vi "LaneFolower.vi"() -> ()   [LabVIEW 2024]
uses:
  <vilib>/Python/Open Venv Python Session.vi
panel:
  in  "File Path":path
  in  "Lane_No.":i32
  out "ToGoLane_X":dbl[](array[numeric])=[-0.009502511471509933, -0.00958104245364666, -0.009974642656743526, -0.010631692595779896, -0.011504605412483215, -0.01254978682845831, -0.013727571815252304, -0.015002261847257614, -0.016342105343937874, -0.017719069495797157, -0.019109033048152924, -0.020491652190685272, -0.02185027115046978, -0.023171929642558098, -0.02444736659526825, -0.025670843198895454, -0.026840148493647575, -0.027956662699580193, -0.02902509644627571, -0.030053474009037018, -0.03105323575437069, -0.032038867473602295, -0.03302808105945587, -0.034041572362184525, -0.035102952271699905, -0.036238763481378555, -0.03747819736599922, -0.03885306790471077, -0.04039765149354935, -0.042148612439632416, -0.044144876301288605, -0.04642732813954353, -0.049038924276828766, -0.05202410742640495, -0.05542914569377899, -0.05930148437619209, -0.06368973851203918, -0.06864342093467712, -0.0742126852273941, -0.08044812828302383, -0.08740027993917465, -0.09511960297822952, -0.10365574806928635, -0.11305739730596542, -0.12337195128202438, -0.13464458286762238, -0.1469181925058365, -0.16023248434066772, -0.1746234893798828, -0.190122589468956]
  out "ToGpLane_Y":dbl[](array[numeric])=[0.056673385202884674, 0.06285841017961502, 0.06917627155780792, 0.07562797516584396, 0.08221480250358582, 0.08893834054470062, 0.09580045938491821, 0.10280333459377289, 0.1099495217204094, 0.11724183708429337, 0.1246834471821785, 0.13227789103984833, 0.14002907276153564, 0.14794126152992249, 0.15601910650730133, 0.16426768898963928, 0.17269249260425568, 0.18129947781562805, 0.190094992518425, 0.19908587634563446, 0.208279550075531, 0.2176838517189026, 0.22730717062950134, 0.23715846240520477, 0.24724726378917694, 0.25758373737335205, 0.2681786119937897, 0.27904340624809265, 0.290190190076828, 0.3016318380832672, 0.31338199973106384, 0.32545506954193115, 0.3378663659095764, 0.3506320118904114, 0.3637691140174866, 0.37729573249816895, 0.39123091101646423, 0.4055948555469513, 0.42040887475013733, 0.43569549918174744, 0.4514785706996918, 0.4677831828594208, 0.48463597893714905, 0.5020650625228882, 0.5201000571250916, 0.538772463798523, 0.5581153631210327, 0.5781639218330383, 0.5989552140235901, 0.620528519153595]
  out "Tracking_Err(m)":dbl=0.05746451352461557
  in  "Ld(m)":dbl=1.0 format="%#_13g"
  out "GPS_Steer_CMD(Deg)":dbl=-13.889371307932791
  out "Lane":T1(graph)=[{"Third_Lane_X"=[-0.0093022920191288, -0.009425072930753231, -0.00985750462859869, -0.010548070073127747, -0.011449389159679413, -0.012518086470663548, -0.013714795000851154, -0.015004051849246025, -0.016354387626051903, -0.01773810014128685, -0.01913149282336235, -0.020514462143182755, -0.0218708086758852, -0.023187965154647827, -0.024457033723592758, -0.025672709569334984, -0.026833219453692436, -0.027940329164266586, -0.028999147936701775, -0.03001815639436245, -0.03100910596549511, -0.031986892223358154, -0.03296966105699539, -0.03397832438349724, -0.035036876797676086, -0.03617206588387489, -0.03741329908370972, -0.03879253566265106, -0.04034423828125, -0.04210503771901131, -0.04411381483078003, -0.04641137272119522, -0.04904036968946457, -0.05204509198665619, -0.055471181869506836, -0.05936558172106743, -0.06377621740102768, -0.06875165551900864, -0.07434111088514328, -0.0805937796831131, -0.08755884319543839, -0.09528496116399765, -0.103819839656353, -0.11321000009775162, -0.12350000441074371, -0.13473232090473175, -0.14694637060165405, -0.16017811000347137, -0.17445921897888184, -0.18981638550758362], "Third_Lane_Y"=[0.056663379073143005, 0.06285057216882706, 0.06917034834623337, 0.07562372088432312, 0.08221197873353958, 0.0889367088675499, 0.09579980373382568, 0.10280342400074005, 0.10995016992092133, 0.11724283546209335, 0.124684639275074, 0.13227911293506622, 0.140030175447464, 0.14794212579727173, 0.15601962804794312, 0.16426779329776764, 0.17269212007522583, 0.18129855394363403, 0.190093532204628, 0.19908387959003448, 0.20827704668045044, 0.21768087148666382, 0.22730378806591034, 0.2371547818183899, 0.24724338948726654, 0.2575797736644745, 0.2681747376918793, 0.27903974056243896, 0.29018694162368774, 0.3016291558742523, 0.31338009238243103, 0.32545405626296997, 0.3378664553165436, 0.3506333529949188, 0.36377182602882385, 0.37729987502098083, 0.3912365734577179, 0.40560200810432434, 0.420417457818985, 0.4357053339481354, 0.4514893889427185, 0.4677945673465729, 0.4846474230289459, 0.5020757913589478, 0.520109236240387, 0.5387787818908691, 0.5581173896789551, 0.5781599283218384, 0.5989429354667664, 0.6205053329467773]}, {"Third_Lane_X"=[0.4193677306175232, 0.4193677306175232, 0.4193677306175232, 0.4193677306175232, 0.4193677306175232, 0.4193677306175232, 0.4193677306175232, 0.4193677306175232, 0.4193677306175232, 0.42097243201055806, 0.42392416776651465, 0.42498393701902, 0.4250357962365585, 0.4243763465398626, 0.4232724906954244, 0.42195267611738735, 0.42051152778688927, 0.4190382473884229, 0.4175688753060556, 0.4161152139823713, 0.4146708213415447, 0.41321472214946825, 0.41172401655332985, 0.41016610607672, 0.40850818978861925, 0.4067346649283272, 0.4047908396323909, 0.4026850775517133, 0.4003864312158304, 0.3978821262918225, 0.3951741967138616, 0.3922227445599256, 0.38908504618485606, 0.3857545290688188, 0.3822306560533131, 0.37854025974870753, 0.37470173287875413, 0.3707522348284704, 0.36670607410360523, 0.362607736842811, 0.3584846745888019, 0.35437860537888727, 0.3503258684770675, 0.3463709544143118, 0.3441532850265503, 0.3441532850265503, 0.3441532850265503, 0.3441532850265503, 0.3441532850265503, 0.3441532850265503], "Third_Lane_Y"=[0.056663379073143005, 0.06867623572446863, 0.08068909237579423, 0.09270194902711985, 0.10471480567844546, 0.11672766232977108, 0.1287405189810967, 0.1407533756324223, 0.15276623228374792, 0.16477908893507354, 0.17679194558639916, 0.18880480223772478, 0.2008176588890504, 0.21283051554037602, 0.2248433721917016, 0.23685622884302723, 0.24886908549435285, 0.2608819421456785, 0.27289479879700407, 0.2849076554483297, 0.2969205120996553, 0.30893336875098093, 0.32094622540230655, 0.33295908205363217, 0.3449719387049578, 0.3569847953562834, 0.36899765200760903, 0.3810105086589346, 0.3930233653102602, 0.40503622196158584, 0.41704907861291146, 0.4290619352642371, 0.4410747919155627, 0.4530876485668883, 0.46510050521821394, 0.47711336186953957, 0.4891262185208652, 0.5011390751721908, 0.5131519318235164, 0.525164788474842, 0.5371776451261676, 0.5491905017774932, 0.5612033584288189, 0.5732162150801444, 0.5852290717314701, 0.5972419283827957, 0.6092547850341213, 0.6212676416854469, 0.6332804983367726, 0.6452933549880981]}, {"Third_Lane_X"=[0.0, 0.0, 0.0, 0.0, 0.0, 0.0, 0.0, 0.0, 0.0, 0.0, 0.0, 0.0, 0.0, 0.0, 0.0, 0.0, 0.0, 0.0, 0.0, 0.0, 0.0, 0.0, 0.0, 0.0, 0.0, 0.0, 0.0, 0.0, 0.0, 0.0, 0.0, 0.0, 0.0, 0.0, 0.0, 0.0, 0.0, 0.0, 0.0, 0.0, 0.0, 0.0, 0.0, 0.0, 0.0, 0.0, 0.0, 0.0, 0.0, 0.0], "Third_Lane_Y"=[0.0, 0.0, 0.0, 0.0, 0.0, 0.0, 0.0, 0.0, 0.0, 0.0, 0.0, 0.0, 0.0, 0.0, 0.0, 0.0, 0.0, 0.0, 0.0, 0.0, 0.0, 0.0, 0.0, 0.0, 0.0, 0.0, 0.0, 0.0, 0.0, 0.0, 0.0, 0.0, 0.0, 0.0, 0.0, 0.0, 0.0, 0.0, 0.0, 0.0, 0.0, 0.0, 0.0, 0.0, 0.0, 0.0, 0.0, 0.0, 0.0, 0.0]}]
  out "Third_Lane_X":dbl[](array[numeric])
  out "Third_Lane_Y":dbl[](array[numeric])
  out "Second_Lane_X":dbl[](array[numeric])=[0.4193677306175232, 0.4193677306175232, 0.4193677306175232, 0.4193677306175232, 0.4193677306175232, 0.4193677306175232, 0.4193677306175232, 0.4193677306175232, 0.4193677306175232, 0.42097243201055806, 0.42392416776651465, 0.42498393701902, 0.4250357962365585, 0.4243763465398626, 0.4232724906954244, 0.42195267611738735, 0.42051152778688927, 0.4190382473884229, 0.4175688753060556, 0.4161152139823713, 0.4146708213415447, 0.41321472214946825, 0.41172401655332985, 0.41016610607672, 0.40850818978861925, 0.4067346649283272, 0.4047908396323909, 0.4026850775517133, 0.4003864312158304, 0.3978821262918225, 0.3951741967138616, 0.3922227445599256, 0.38908504618485606, 0.3857545290688188, 0.3822306560533131, 0.37854025974870753, 0.37470173287875413, 0.3707522348284704, 0.36670607410360523, 0.362607736842811, 0.3584846745888019, 0.35437860537888727, 0.3503258684770675, 0.3463709544143118, 0.3441532850265503, 0.3441532850265503, 0.3441532850265503, 0.3441532850265503, 0.3441532850265503, 0.3441532850265503]
  out "Second_Lane_Y":dbl[](array[numeric])=[0.056663379073143005, 0.06867623572446863, 0.08068909237579423, 0.09270194902711985, 0.10471480567844546, 0.11672766232977108, 0.1287405189810967, 0.1407533756324223, 0.15276623228374792, 0.16477908893507354, 0.17679194558639916, 0.18880480223772478, 0.2008176588890504, 0.21283051554037602, 0.2248433721917016, 0.23685622884302723, 0.24886908549435285, 0.2608819421456785, 0.27289479879700407, 0.2849076554483297, 0.2969205120996553, 0.30893336875098093, 0.32094622540230655, 0.33295908205363217, 0.3449719387049578, 0.3569847953562834, 0.36899765200760903, 0.3810105086589346, 0.3930233653102602, 0.40503622196158584, 0.41704907861291146, 0.4290619352642371, 0.4410747919155627, 0.4530876485668883, 0.46510050521821394, 0.47711336186953957, 0.4891262185208652, 0.5011390751721908, 0.5131519318235164, 0.525164788474842, 0.5371776451261676, 0.5491905017774932, 0.5612033584288189, 0.5732162150801444, 0.5852290717314701, 0.5972419283827957, 0.6092547850341213, 0.6212676416854469, 0.6332804983367726, 0.6452933549880981]
  out "First_Lane_Y":dbl[](array[numeric])=[0.056663379073143005, 0.06285057216882706, 0.06917034834623337, 0.07562372088432312, 0.08221197873353958, 0.0889367088675499, 0.09579980373382568, 0.10280342400074005, 0.10995016992092133, 0.11724283546209335, 0.124684639275074, 0.13227911293506622, 0.140030175447464, 0.14794212579727173, 0.15601962804794312, 0.16426779329776764, 0.17269212007522583, 0.18129855394363403, 0.190093532204628, 0.19908387959003448, 0.20827704668045044, 0.21768087148666382, 0.22730378806591034, 0.2371547818183899, 0.24724338948726654, 0.2575797736644745, 0.2681747376918793, 0.27903974056243896, 0.29018694162368774, 0.3016291558742523, 0.31338009238243103, 0.32545405626296997, 0.3378664553165436, 0.3506333529949188, 0.36377182602882385, 0.37729987502098083, 0.3912365734577179, 0.40560200810432434, 0.420417457818985, 0.4357053339481354, 0.4514893889427185, 0.4677945673465729, 0.4846474230289459, 0.5020757913589478, 0.520109236240387, 0.5387787818908691, 0.5581173896789551, 0.5781599283218384, 0.5989429354667664, 0.6205053329467773]
  out "First_Lane_X":dbl[](array[numeric])=[-0.0093022920191288, -0.009425072930753231, -0.00985750462859869, -0.010548070073127747, -0.011449389159679413, -0.012518086470663548, -0.013714795000851154, -0.015004051849246025, -0.016354387626051903, -0.01773810014128685, -0.01913149282336235, -0.020514462143182755, -0.0218708086758852, -0.023187965154647827, -0.024457033723592758, -0.025672709569334984, -0.026833219453692436, -0.027940329164266586, -0.028999147936701775, -0.03001815639436245, -0.03100910596549511, -0.031986892223358154, -0.03296966105699539, -0.03397832438349724, -0.035036876797676086, -0.03617206588387489, -0.03741329908370972, -0.03879253566265106, -0.04034423828125, -0.04210503771901131, -0.04411381483078003, -0.04641137272119522, -0.04904036968946457, -0.05204509198665619, -0.055471181869506836, -0.05936558172106743, -0.06377621740102768, -0.06875165551900864, -0.07434111088514328, -0.0805937796831131, -0.08755884319543839, -0.09528496116399765, -0.103819839656353, -0.11321000009775162, -0.12350000441074371, -0.13473232090473175, -0.14694637060165405, -0.16017811000347137, -0.17445921897888184, -0.18981638550758362]
  out "ImageString":string
  out "error out":errorcluster
  out "Python Loop Process Time":u32=33
  in  "stop":bool
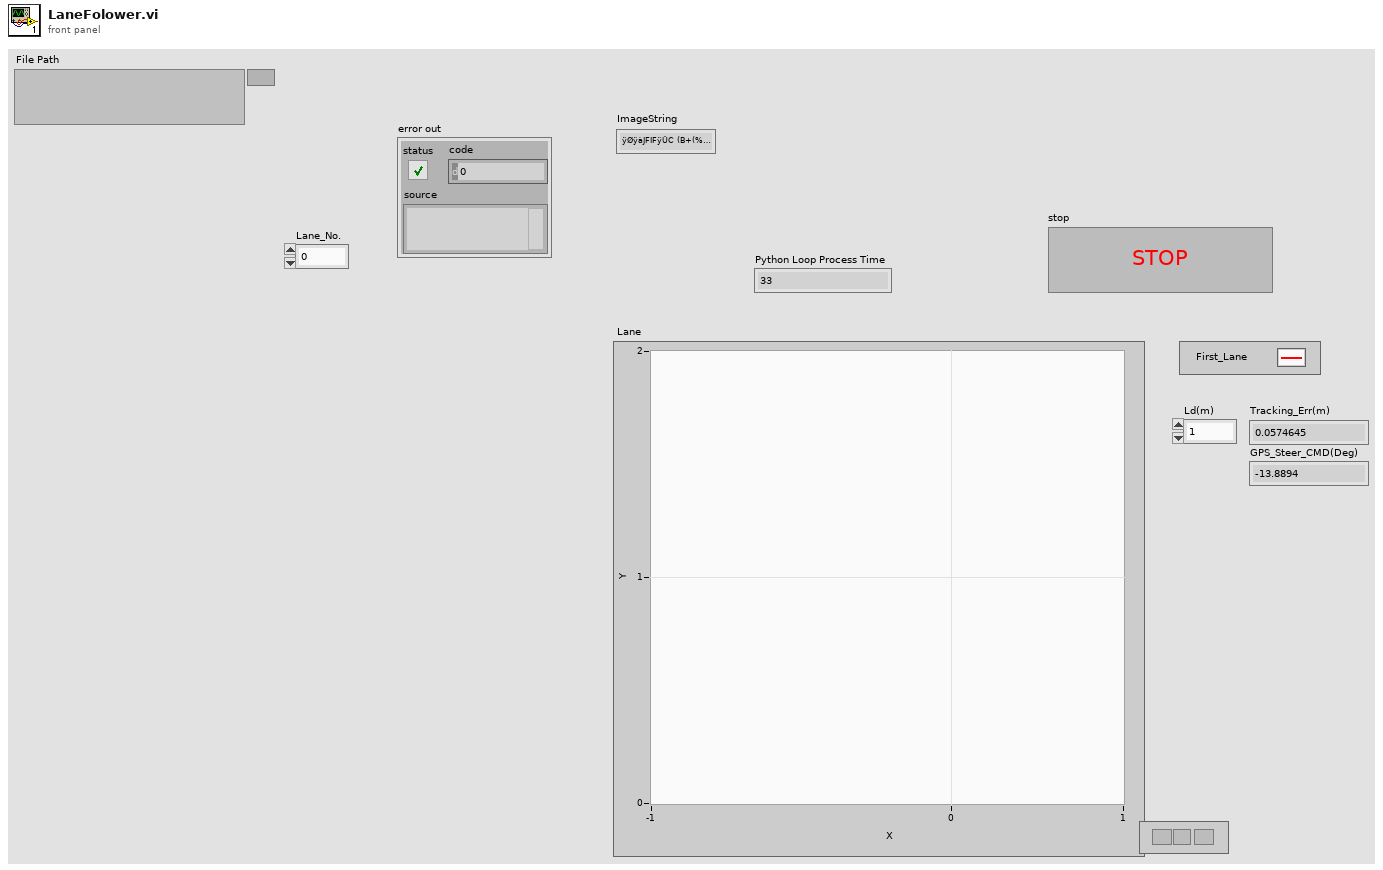
[diagram p1: front panel]
types:
  T1 = cluster{"Third_Lane_X":dbl[], "Third_Lane_Y":dbl[]}[]
  T2 = typedef "IMAQ Image.ctl" = refnum<image>
  T3 = cluster{"First_Lane_X":dbl[], "First_Lane_Y":dbl[]}
  T4 = cluster{"Second_Lane_X":dbl[], "Second_Lane_Y":dbl[]}
  T5 = cluster{"Third_Lane_X":dbl[], "Third_Lane_Y":dbl[]}
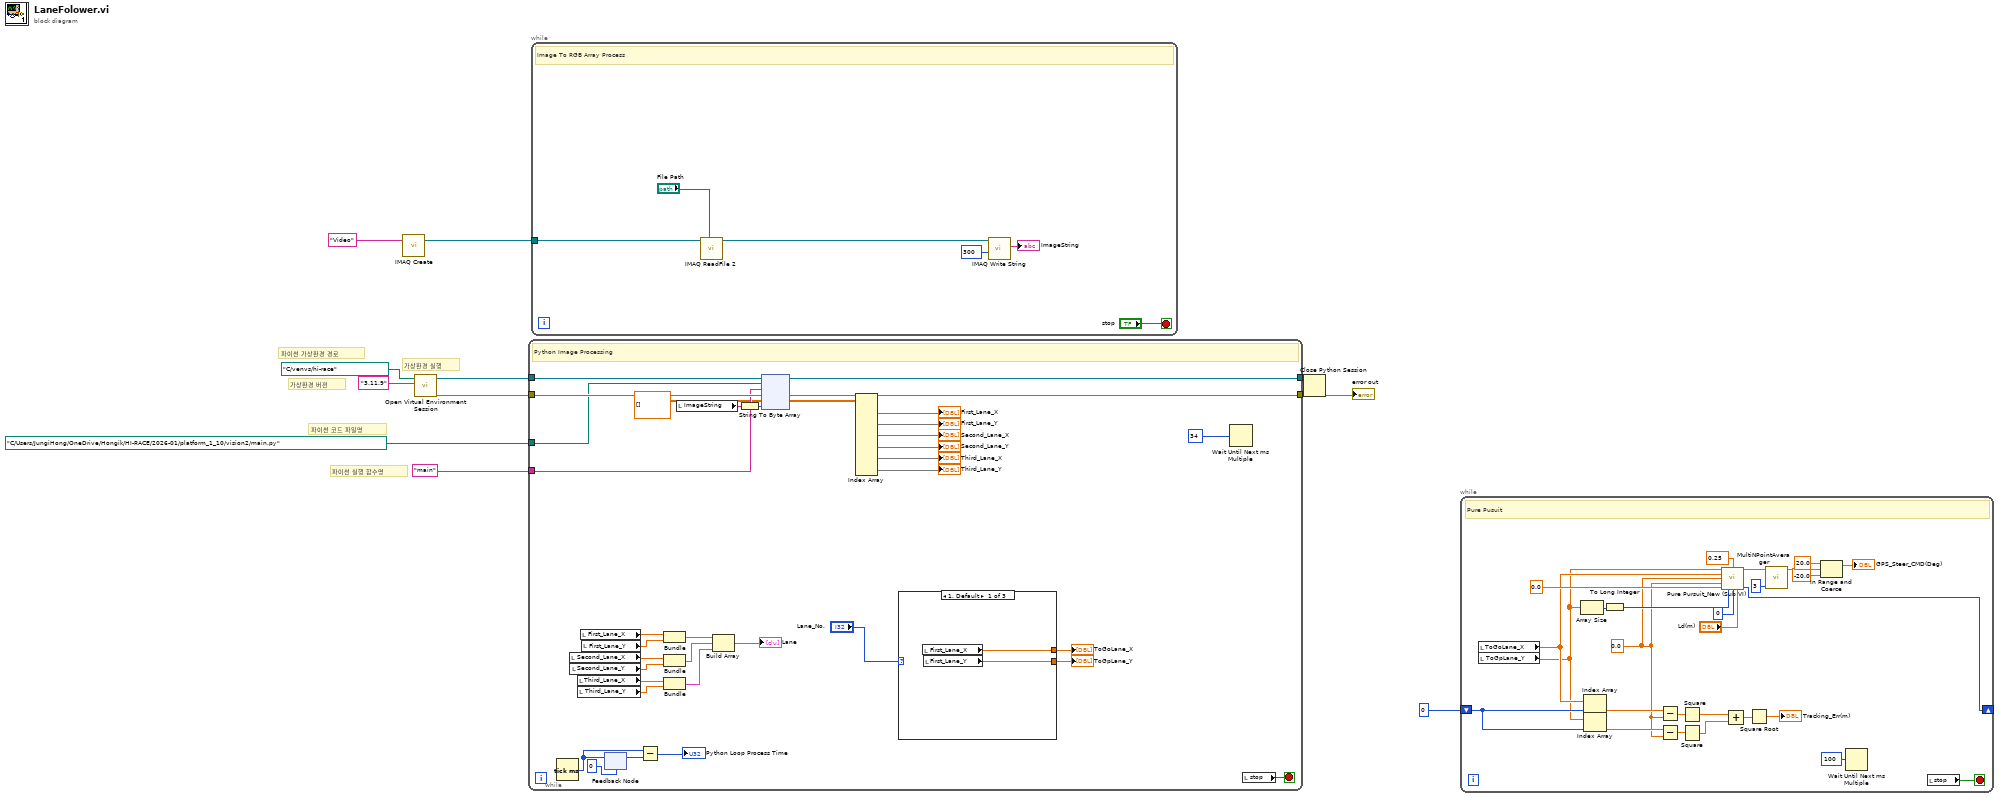
[diagram p0: block diagram]
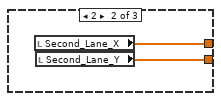
[diagram p2: hidden frame]
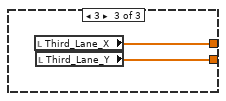
[diagram p3: hidden frame]
diagram:
  # "파이썬 실행 함수명"
  # "파이썬 코드 파일명"
  # "가상환경 실행"
  # "가상환경 버젼"
  # "파이썬 가상환경 경로"
  n1 = call "IMAQ Create"("Image Name"="Video") -> ("New Image"=w10:T2)  [unwired: 4 in, 1 out]
  n2 = call-poly <vilib>:"Open Virtual Environment Session.vi"("Python version"="3.11.9", "Env path"=path "C:/venvs/hi-race") -> ("error out"=w6:errorcluster, "session out"=w7:refnum<k35>)  [unwired: 8 in]
  n3 = while {
    tunnel: path "C:/Users/JungiHong/OneDrive/Hongik/HI-RACE/2026-01/platform_1_10/vision2/main.py" ("Name") -> [w43]
    tunnel: "main" ("module out") -> [w42]
    tunnel: w7 -> [w45]
    tunnel: [w47] -> w9
    tunnel: w6 -> [w44]
    tunnel: [w46] -> w8
    stop <- w41 stop-if-true
    # "Python Image Processing"
    n4 = Tick Count (ms)() -> (millisecond timer value=w37:u32)
    n5 = local read "Second_Lane_X"() -> (w26:dbl[])
    n6 = local read "Second_Lane_Y"() -> (w25:dbl[])
    n7 = local read "Third_Lane_X"() -> (w24:dbl[])
    n8 = local read "Third_Lane_Y"() -> (w23:dbl[])
    n9 = local read "First_Lane_X"() -> (w28:dbl[])
    n10 = local read "First_Lane_Y"() -> (w27:dbl[])
    n11 = feedback #1(u32 0 ("millisecond timer value")) -> (w38:u32)
    n12 = feedback-in #1(w37) -> ()
    n13 = Subtract(x=w37, y=w38) -> (x-y=→"Python Loop Process Time":u32)
    n14 = Bundle("First_Lane_X"=w28, "First_Lane_Y"=w27) -> (w22:T3)  [unwired: 1 in]
    n15 = Bundle("Second_Lane_X"=w26, "Second_Lane_Y"=w25) -> (w21:T4)  [unwired: 1 in]
    n16 = Bundle("Third_Lane_X"=w24, "Third_Lane_Y"=w23) -> (w20:T5)  [unwired: 1 in]
    n17 = local read "ImageString"() -> (w36:string)
    n18 = Build Array(w22, w21, w20) -> (→"Lane":T1)
    n19 = String To Byte Array(string=w36) -> (unsigned byte array=w35:u8[])
    n20 = node(w45, w43, w42, w44, dbl[][] [] ("appended array"), w35) -> (w47:refnum<k35>, w46:errorcluster, w14:dbl[][])  [unwired: 1 in, 2 out]
    n21 = Index Array(array=w14) -> (element #1=→"First_Lane_X":dbl[], element #2=→"First_Lane_Y":dbl[], element #3=→"Second_Lane_X":dbl[], element #4=→"Second_Lane_Y":dbl[], element #5=→"Third_Lane_X":dbl[], element #6=→"Third_Lane_Y":dbl[])  [unwired: 12 in]
    n22 = case shown="1, Default" "Lane_No." {
      tunnel: [w49 w51 w53] -> w17
      tunnel: [w48 w50 w52] -> w16
      frame 1, Default {
        n23 = local read "First_Lane_X"() -> (w49:dbl[])
        n24 = local read "First_Lane_Y"() -> (w48:dbl[])
      }
      frame 2 {
        n25 = local read "Second_Lane_X"() -> (w51:dbl[])
        n26 = local read "Second_Lane_Y"() -> (w50:dbl[])
      }
      frame 3 {
        n27 = local read "Third_Lane_X"() -> (w53:dbl[])
        n28 = local read "Third_Lane_Y"() -> (w52:dbl[])
      }
    }
    "ToGoLane_X" <- w17
    "ToGpLane_Y" <- w16
    n29 = Wait Until Next ms Multiple(millisecond multiple=u32 34) -> ()  [unwired: 1 out]
    n30 = local read "stop"() -> (w41:bool)
  }
  n31 = while {
    tunnel: w10 -> [w56]
    stop <- "stop" stop-if-true
    # "Image To RGB Array Process"
    n32 = call "IMAQ ReadFile 2"("File Path"="File Path", "Image"=w56) -> ("Image Out"=w55:T2)  [unwired: 5 in, 4 out]
    n33 = call-poly "IMAQ Write String"("Image Quality"=u32 300, "Image"=w55) -> ("FileString"=→"ImageString":string)  [unwired: 7 in, 2 out]
  }
  n34 = Close Python Session(session in=w9, error in=w8) -> (11:→"error out":errorcluster)
  n35 = while {
    shift-right: [w86] -> _
    shift-left: 0 ("Index(near vehicle)") -> [w85]
    stop <- w84 stop-if-true
    w60 = 0.0 ("Y_Current")
    # "Pure Pusuit"
    n36 = local read "ToGoLane_X"() -> (w62:dbl[])
    n37 = local read "ToGpLane_Y"() -> (w61:dbl[])
    n38 = Array Size(array=w61) -> (size(s)=w71:i32)
    n39 = Index Array(array=w62, index=w85) -> (element=w82:dbl)
    n40 = Index Array(array=w61, index=w85) -> (element=w83:dbl)
    n41 = To Long Integer(number=w71) -> (32bit integer=w70:i32)
    n42 = Subtract(x=w82, y=w60) -> (x-y=w77:dbl)
    n43 = Subtract(x=w83, y=w60) -> (x-y=w76:dbl)
    n44 = Square(x=w77) -> (x^2=w75:dbl)
    n45 = Square(x=w76) -> (x^2=w74:dbl)
    n46 = call "Pure Pursuit_New (Sub VI).vi"("x_lat_path"=w61, "L"=0.25, "y_long_path"=w62, "X_Current"=w60, "Y_Current"=w60, "Heading_Current"=0.0, "#pnt"=w70, "WP no_pre"=0, "LAD"="Ld(m)") -> ("Steer_CMD(Deg)"=w66:dbl, "Index(near vehicle)"=w86:i32)  [unwired: 3 in, 2 out]
    n47 = Add(x=w75, y=w74) -> (x+y=w73:dbl)
    n48 = Square Root(x=w73) -> (sqrt(x)=→"Tracking_Err(m)":dbl)
    n49 = call "MultiNPointAverager.vi"("N point average"=3 ("WP no_pre"), "Data_input"=w66) -> ("숫자형"=w81:dbl)  [unwired: 9 in]
    n50 = In Range and Coerce(upper limit=20.0, x=w81, lower limit=-20.0) -> (coerced(x)=→"GPS_Steer_CMD(Deg)":dbl)  [unwired: 1 out]
    n51 = Wait Until Next ms Multiple(millisecond multiple=u32 100 ("ms 배수")) -> ()  [unwired: 1 out]
    n52 = local read "stop"() -> (w84:bool)
  }
